vi "to string.vi"(8 "error in":errorcluster, 11 "Simple Sequencer TBM configuration in":refnum<class "Simple Sequencer TBM configuration.lvclass">) -> (0 "error out":errorcluster, 1 "data":string, 2 "version":string, 3 "Simple Sequencer TBM configuration out":refnum<class "Simple Sequencer TBM configuration.lvclass">)   [LabVIEW 2015, in "Simple Sequencer TBM configuration.lvclass"]
doc: "Provides an interface for saving a module configuration to a file or other serialized data source. It is recommended that all children of this class store data in two sets--data required for its own initialization, and any data required for parent initialization--and that each implementation uses the <b>Call Parent Method</b> primitive to serialize parent information."
uses:
  Simple Sequencer TBM configuration.lvclass
  Simple Sequencer TBM configuration.lvclass/Simple Sequencer TBM configuration.ctl
  current version.vi
  sequencer parent classes/sequencer config parent/base TBM sequencer configuration.lvclass
  sequencer parent classes/action configuration parent/action configuration.lvclass
  <vilib>/NI/Configuration Framework/serializable configuration/NISE_CEF_serializable configuration.lvclass
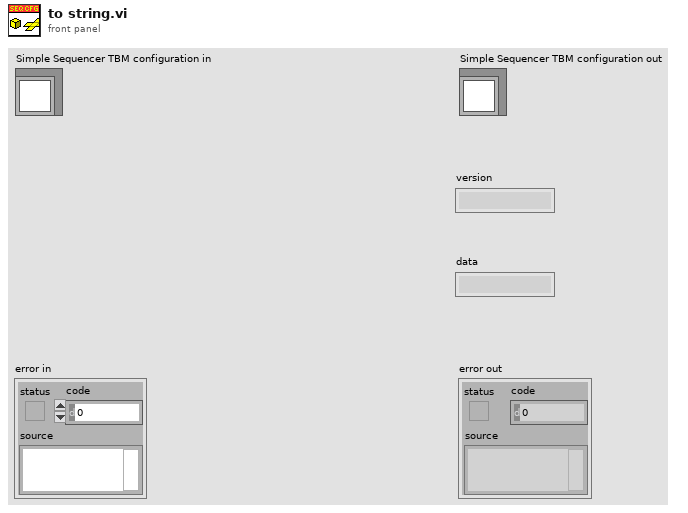
[diagram p1: front panel]
types:
  T1 = typedef "Simple Sequencer TBM configuration.lvclass/sequence definition.ctl" = cluster{"sequence name":string, "action configs":refnum<class "action configuration.lvclass">[]}
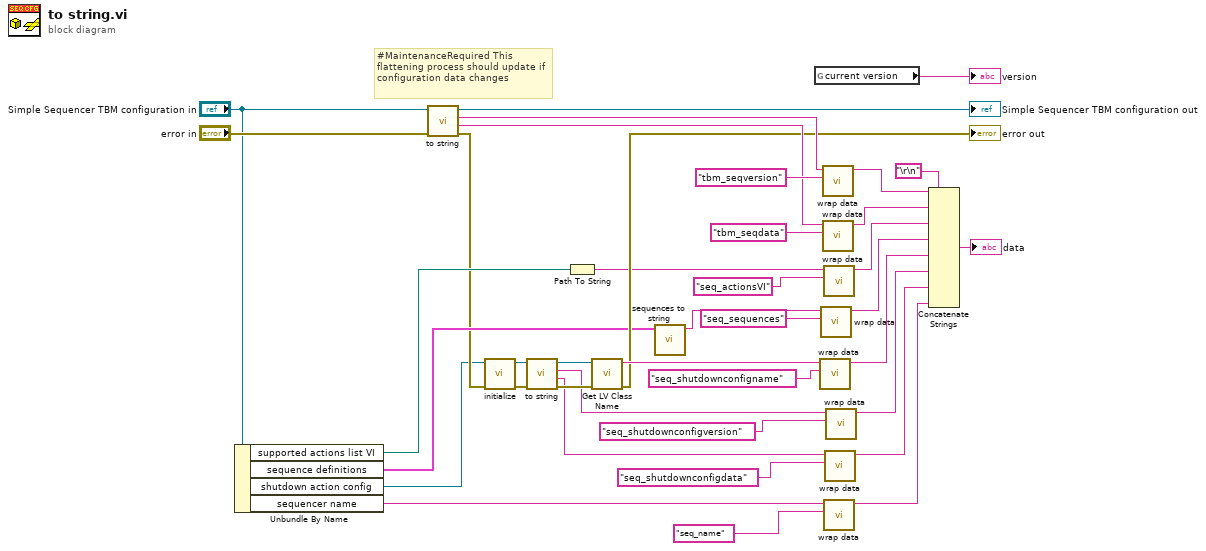
[diagram p0: block diagram]
diagram:
  w7 = "\r\n"
  # "#MaintenanceRequired This flattening process should update if configuration data changes"
  n1 = Unbundle By Name("Simple Sequencer TBM configuration in") -> ("supported actions list VI"=w6:path, "sequence definitions"=w11:T1[], "shutdown action config"=w1:refnum<class "action configuration.lvclass">, "sequencer name"=w23:string)
  n2 = call-parent "to string.vi"("error in"="error in", "engine configuration in"="Simple Sequencer TBM configuration in") -> ("error out"=w2:errorcluster, "data"=w31:string, "version"=w32:string, "engine configuration out"=→"Simple Sequencer TBM configuration out":refnum<class "Simple Sequencer TBM configuration.lvclass">)  [unwired: 6 in]
  n3 = call <vilib>:"initialize.vi"("error in"=w2, "configuration in"=w1) -> ("error out"=w3:errorcluster, "configuration out"=w4:refnum<class "action configuration.lvclass">)  [unwired: 7 in, 1 out]
  n4 = call-dynamic "to string.vi"("error in"=w3, "configuration in"=w4) -> ("error out"=w17:errorcluster, "data"=w14:string, "version"=w15:string, "configuration out"=w18:refnum<class "action configuration.lvclass">)  [unwired: 6 in]
  n5 = Path To String(path=w6) -> (string=w5:string)
  n6 = call <vilib>:"Get LV Class Name.vi"("error in (no error)"=w17, "object"=w18) -> ("error out"=→"error out":errorcluster, "class name"=w21:string)  [unwired: 8 in]
  n7 = call "sequences to string.vi"("sequence definitions"=w11) -> ("string"=w10:string)  [unwired: 10 in]
  n8 = global read "current version.vi" "current version"() -> (→"version":string)
  n9 = call <vilib>:"wrap data.vi"("identifier"="seq_shutdownconfigname", "data to wrap"=w21) -> ("wrapped data"=w13:string)  [unwired: 9 in]
  n10 = call <vilib>:"wrap data.vi"("identifier"="seq_sequences", "data to wrap"=w10) -> ("wrapped data"=w26:string)  [unwired: 9 in]
  n11 = call <vilib>:"wrap data.vi"("identifier"="tbm_seqversion" ("additional identifier"), "data to wrap"=w32) -> ("wrapped data"=w34:string)  [unwired: 9 in]
  n12 = call <vilib>:"wrap data.vi"("identifier"="tbm_seqdata" ("additional identifier"), "data to wrap"=w31) -> ("wrapped data"=w33:string)  [unwired: 9 in]
  n13 = call <vilib>:"wrap data.vi"("identifier"="seq_actionsVI", "data to wrap"=w5) -> ("wrapped data"=w8:string)  [unwired: 9 in]
  n14 = call <vilib>:"wrap data.vi"("identifier"="seq_name", "data to wrap"=w23) -> ("wrapped data"=w22:string)  [unwired: 9 in]
  n15 = call <vilib>:"wrap data.vi"("identifier"="seq_shutdownconfigdata", "data to wrap"=w14) -> ("wrapped data"=w25:string)  [unwired: 9 in]
  n16 = call <vilib>:"wrap data.vi"("identifier"="seq_shutdownconfigversion", "data to wrap"=w15) -> ("wrapped data"=w12:string)  [unwired: 9 in]
  n17 = Concatenate Strings(w34, w7, w33, w7, w8, w7, w26, w7, w13, w7, w12, w7, w25, w7, w22) -> (→"data":string)
